vi "Single Tone Audio Measurements (N Ch).vi"(6 "units settings":T2, 8 "error in":errorcluster, 10 "measurement settings":T5={"Band start"=20.0, "Band stop"=20000.0, "Amplitude"=1.0, "Frequency"=1000.0, "Full scale range"=3.16}, 11 "waveforms":waveform(dbl)[](array[waveform])) -> (0 "error out":errorcluster, 1 "spectra":cluster{"x0":dbl, "dx":dbl, "magnitude":dbl[]}[](array[cluster]), 2 "waveforms":waveform(dbl)[](array[waveform]), 3 "results":T1[](array[typedef]))   [LabVIEW 2021]
uses:
  controls/single tone audio measurement settings.ctl
  controls/units settings.ctl
  controls/units - snr.ctl
  controls/units - ratio.ctl
  controls/single tone audio measurements.ctl
  <vilib>/addons/_NISVFA/_Shared subVIs/Common/SVL Set dB Reference (N Ch - 1 Ref).vi
  <vilib>/addons/Sound and Vibration/svt_Single Tone Measurements/SVT Spurious Free Dynamic Range (Frequency) (1 Ch).vi
  <vilib>/addons/_NISVFA/_Spectrum Processing/SVFA Unit Conversion (Complex) (1 Ch).vi
  <vilib>/addons/_NISVFA/_Shared subVIs/Common/SVL Set dB Reference (1 Ch).vi
  <vilib>/addons/_NISVFA/_Spectrum Processing/SVFA Get Spectrum Subset.vi
  <vilib>/addons/_NISVFA/_Spectrum Processing/SVFA Get Spectrum Subset (Complex) (1 Ch).vi
  <vilib>/addons/_NISVFA/_Shared subVIs/Common/svc_Window Parameters.vi
  <vilib>/addons/_NISVFA/_Shared subVIs/Common/svc_Extract Single Tone Information (complex).vi
  <vilib>/addons/_NISVFA/_Shared subVIs/Common/svc_Check Frequency Range in Spectrum.vi
  <vilib>/addons/_NISVFA/_Spectrum Processing/SVFA Spectrum Peak Search.vi
  <vilib>/addons/_NISVFA/_Spectrum Processing/SVFA Spectrum Peak Search (1 Ch).vi
  <vilib>/addons/_NISVFA/_Shared subVIs/Common/svc_Spectrum Units.vi
  <vilib>/addons/_NISVFA/_Shared subVIs/Common/svc_Log View for Spectrum (1Ch).vi
  <vilib>/addons/_NISVFA/_Spectrum Processing/SVFA Unit Conversion (1 Ch).vi
  <vilib>/addons/_NISVFA/_Shared subVIs/Common/svc_Complex Datatype Defaults.vi
  <vilib>/addons/_NISVFA/_Shared subVIs/Common/SVL Set dB Reference (variant).vi
  <vilib>/addons/_NISVFA/_Shared subVIs/Common/svc_Build Unit Label for Frequency Range.vi
  <vilib>/addons/_NISVFA/_Spectrum Processing/SVFA Get Tone Amplitude and Phase (1 Ch).vi
  <vilib>/addons/_NISVFA/_Spectrum Processing/subVIs/svfa_Compute Complex Spectrum for Export.vi
  <vilib>/addons/_NISVFA/_Shared subVIs/Common/svc_Check Frequency Range in Bandwidth.vi
  <vilib>/addons/_NISVFA/_Shared subVIs/Common/svc_Convert Start and Stop to Start Index and Length.vi
  <vilib>/addons/_NISVFA/_Spectrum Processing/subVIs/svfa_Spectrum Peak Search.vi
  <vilib>/addons/_NISVFA/_Shared subVIs/Common/svc_Format Value (DBL).vi
  <vilib>/addons/_NISVFA/_Shared subVIs/Common/svc_Get Weighting Enum and Labels.vi
  <vilib>/addons/_NISVFA/_Shared subVIs/Common/svc_Engineering Units to Unit Label.vi
  <vilib>/addons/_NISVFA/_Shared subVIs/Common/svc_Surround NonAlpha String with Parentheses.vi
  <vilib>/dlg_ctls.llb/Space Constant.vi
  <vilib>/addons/_NISVFA/_Shared subVIs/Common/svc_Unwrap Phase.vi
  <vilib>/addons/_NISVFA/_Shared subVIs/Common/svc_Convert Spectrum Array to dB.vi
  <vilib>/addons/_NISVFA/_Spectrum Processing/subVIs/svfa_Conversion Utility (spectrum info).vi
  <vilib>/addons/_NISVFA/_Spectrum Processing/subVIs/svfa_Window Frequency Response.vi
  <vilib>/addons/_NISVFA/_Spectrum Processing/subVIs/svfa_Window Frequency Response (double array).vi
  <vilib>/Analysis/baseanly.llb/Dot Product.vi
  <vilib>/Analysis/baseanly.llb/Complex Dot Product.vi
  <vilib>/addons/_NISVFA/_Spectrum Processing/subVIs/svfa_Peak Rough Search Indices.vi
  <vilib>/addons/_NISVFA/_Shared subVIs/Common/svc_Unit Label Lexical Class.vi
  <vilib>/addons/_NISVFA/_Spectrum Processing/subVIs/svfa_Peak to RMS to Peak2Peak.vi
  <vilib>/addons/_NISVFA/_Spectrum Processing/subVIs/svfa_Mag to Mag2.vi
  <vilib>/addons/_NISVFA/_Spectrum Processing/subVIs/svfa_Linear to dB.vi
  <vilib>/addons/_NISVFA/_Spectrum Processing/subVIs/svfa_dBrefA to dBrefB.vi
  <vilib>/addons/_NISVFA/_Spectrum Processing/subVIs/svfa_Spectrum to Spectral Density.vi
  <vilib>/addons/_NISVFA/_Spectrum Processing/subVIs/svfa_Rect Window Frequency Response.vi
  <vilib>/addons/_NISVFA/_Spectrum Processing/subVIs/svfa_Cosine Window Coefficients.vi
  <vilib>/addons/_NISVFA/_Shared subVIs/Common/svc_Caller VI Returned in Error Source.vi
  <vilib>/addons/Sound and Vibration/svt_Single Tone Measurements/SVT Gain (Time) (1 Ch).vi
  <vilib>/addons/Sound and Vibration/svt_Distortion/SVT SNR without Harmonics (Frequency) (1 Ch).vi
  <vilib>/addons/_NISVFA/_Spectrum Processing/SVFA Extract Single Tone Information (Complex) (1 Ch).vi
  <vilib>/addons/Sound and Vibration/svt_Single Tone Measurements/SVT Dynamic Range (Frequency) (1 Ch).vi
  <vilib>/addons/Sound and Vibration/svt_Distortion/subVIs/sv_Check Data Valid (Audio) (1 Ch).vi
  <vilib>/addons/_NISVFA/_Shared subVIs/Common/svc_Convert Frequency to Frequency String.vi
  <vilib>/Analysis/4window.llb/window parameters.vi
  <vilib>/Analysis/4window.llb/Window Properties.vi
  <vilib>/Analysis/4window.llb/Window Properties by Name.vi
  <vilib>/addons/_NISVFA/_Spectrum Processing/subVIs/svfa_Spectrum Peak Tone Search and Estimation (complex).vi
  <vilib>/measure/masignal.llb/Tones and Noise Waveform.vi
  <vilib>/addons/_NISVFA/_Shared subVIs/Common/svc_FFT with Window.vi
  <vilib>/Analysis/1siggen.llb/Square Wave.vi
  <vilib>/addons/_NISVFA/_Spectrum Processing/subVIs/svfa_Three Finger Peak Search.vi
  <vilib>/addons/Sound and Vibration/svt_Distortion/subVIs/sv_Peak View Amplitude (1 Ch).vi
  <vilib>/addons/Sound and Vibration/svt_Single Tone Measurements/SoundVib_SingleTone.lvlib
  <vilib>/addons/Sound and Vibration/svt_Distortion/SoundVib_Distortion.lvlib
  controls/audio controls.lvlib
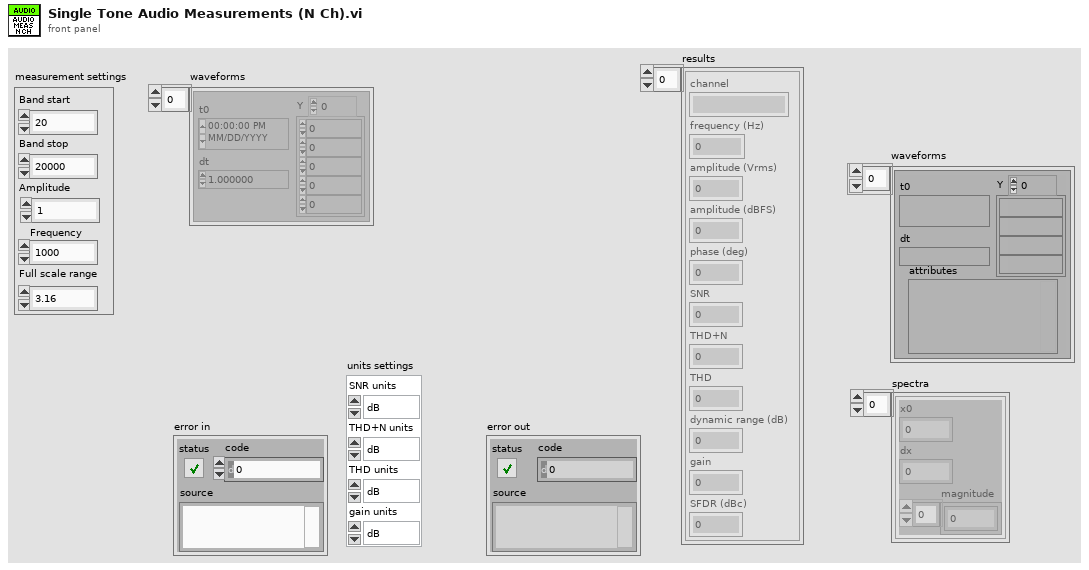
[diagram p1: front panel]
types:
  T1 = typedef "audio controls.lvlib/single tone audio measurements.ctl" = cluster{"channel":string, "frequency (Hz)":dbl, "amplitude (Vrms)":dbl, "amplitude (dBFS)":dbl, "phase (deg)":dbl, "SNR":dbl, "THD+N":dbl, "THD":dbl, "dynamic range (dB)":dbl, "gain":dbl, "SFDR (dBc)":dbl}
  T2 = typedef "audio controls.lvlib/units settings.ctl" = cluster{"SNR units":T3, "THD+N units":T4, "THD units":T4, "gain units":T4}
  T3 = typedef "audio controls.lvlib/units - snr.ctl" = enum32{"dB", "x/y"}
  T4 = typedef "audio controls.lvlib/units - ratio.ctl" = enum32{"dB", "%", "x/y"}
  T5 = typedef "single tone audio measurement settings.ctl" = cluster{"Band start":dbl, "Band stop":dbl, "Amplitude":dbl, "Frequency":dbl, "Full scale range":dbl}
  T6 = cluster{"start frequency":dbl, "stop frequency":dbl}
  T7 = cluster{"SNR units":enum16{"dB", "linear ratio", "%"}, "detected fundamental amplitude units":enum16{"EU rms", "EU peak", "EU peak-peak"}}
  T8 = cluster{"gain units":enum16{"dB", "linear ratio"}, "detected fundamental amplitude units":enum16{"EU rms", "EU peak", "EU peak-peak"}}
  T9 = enum16{"no change", "spectrum", "spectral density"}
  T10 = cluster{"linear/dB":enum16{"no change", "linear", "dB"}, "dB reference (0: no change)":dbl, "power/magnitude":enum16{"no change", "power", "magnitude"}, "view":enum16{"no change", "rms", "peak", "peak-peak"}}
  T11 = typedef "svc_Spectrum Info.ctl" = cluster{"channel name":string, "description":string, "x-axis units":T12, "spectral info":cluster{"spectrum type":T13, "linear/dB":enum16{"linear", "dB"}, "window":u16, "window size":i32, "FFT size":i32}, "engineering units":T14, "custom label":string, "dB reference [EU]":dbl, "peak units":enum16{"rms", "peak", "peak-peak"}, "weighting filter":T15, "spectral density?":bool, "unit label":string, "spectrum skewed?":bool, "complimentary spectrum units":T16}
  T12 = typedef "svc_X-Axis Units.ctl" = u16
  T13 = typedef "svc_Spectrum Type.ctl" = enum16{"FFT Spectrum [complex]", "Amplitude [Magnitude]", "Power [Magnitude^2]", "Cross Spectrum [complex]", "Frequency Response [Complex]"}
  T14 = typedef "svc_Engineering Units Text Ring.ctl" = u16
  T15 = typedef "svc_Weighting Filter Text Ring.ctl" = u16
  T16 = typedef "svc_Complimentary Spectrum Units.ctl" = enum16{"none", "radians", "degrees", "cycles", "imaginary"}
  T17 = cluster{"complex spectrum response":cluster{"f0":dbl, "df":dbl, "complex spectrum":cdb[]}, "spectrum info":T11}
  T18 = cluster{"frequency [Hz]":dbl, "amplitude [EU pk]":dbl, "phase (deg)":dbl}
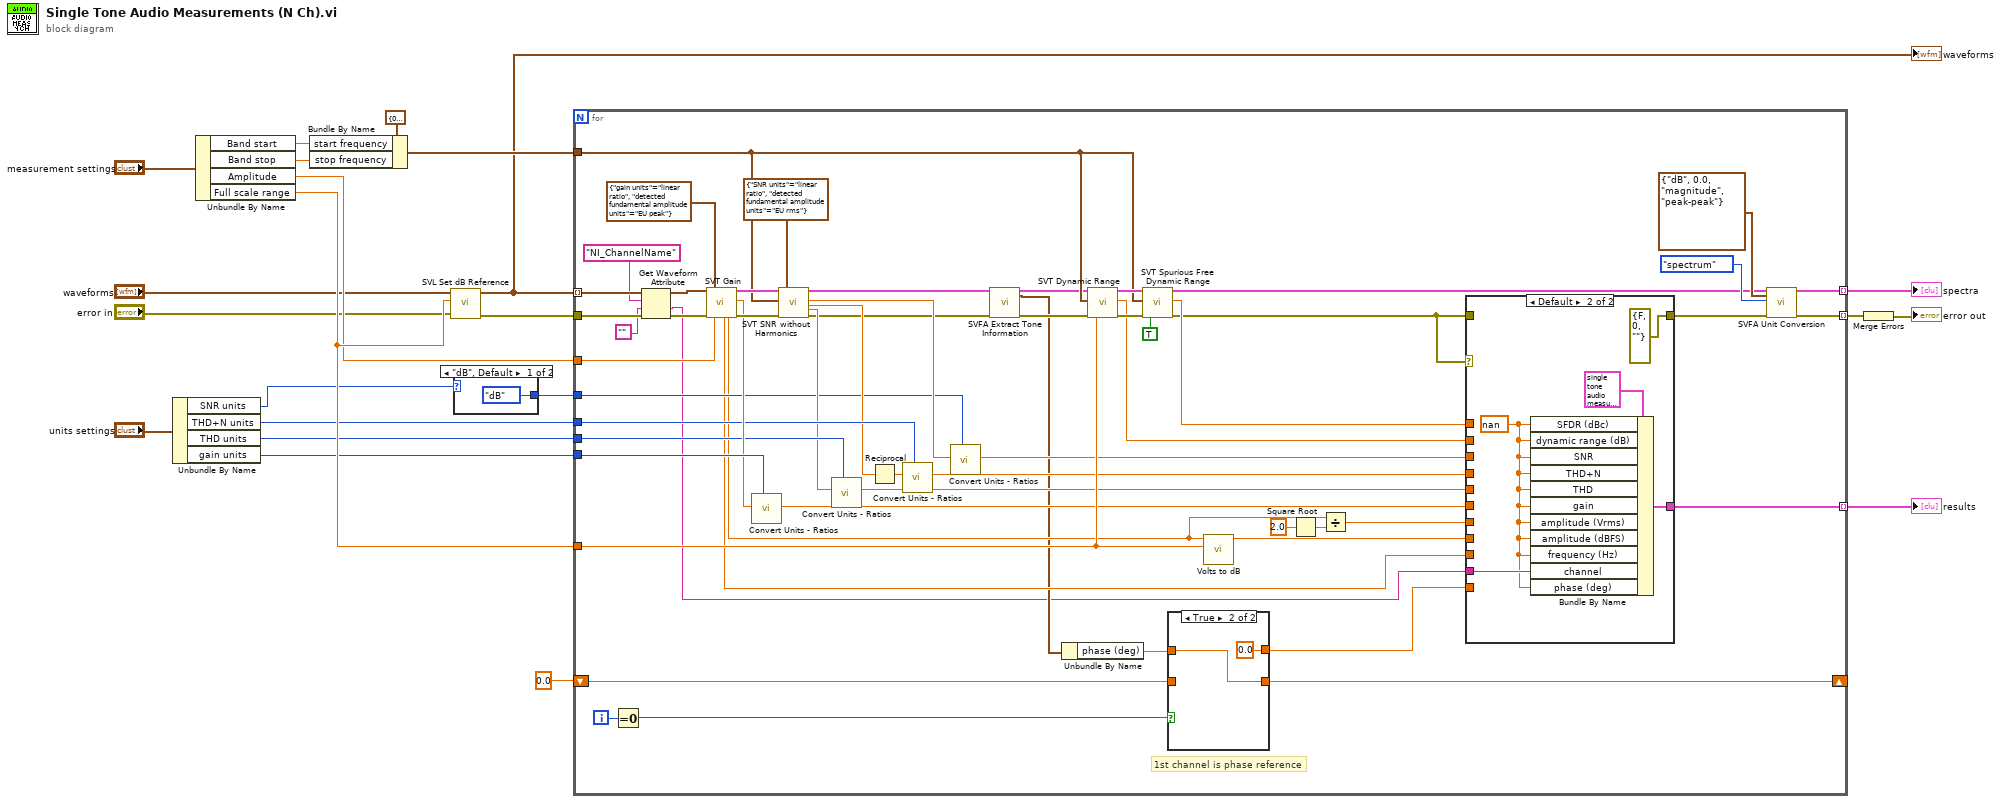
[diagram p0: block diagram]
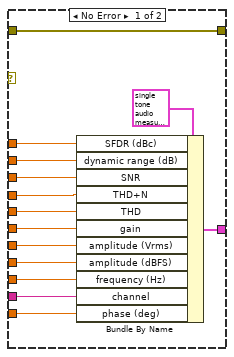
[diagram p2: hidden frame]
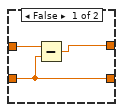
[diagram p3: hidden frame]
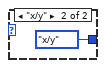
[diagram p4: hidden frame]
diagram:
  n1 = Unbundle By Name("units settings") -> ("SNR units"=w9:T3, "THD+N units"=w11:T4, "THD units"=w10:T4, "gain units"=w12:T4)
  n2 = Unbundle By Name("measurement settings") -> ("Band start"=w21:dbl, "Band stop"=w22:dbl, "Amplitude"=w15:dbl, "Full scale range"=w17:dbl)
  n3 = Bundle By Name(cluster=T6 {"start frequency"=0.0, "stop frequency"=0.0} ("frequency range"), "start frequency"=w21, "stop frequency"=w22) -> (w19:T6)
  n4 = call-poly <vilib>:"SVL Set dB Reference.vi"("error in (no error)"="error in", "dB reference [EU]"=w17, "scaled signals in [EU]"="waveforms") -> ("error out"=w16:errorcluster, "scaled signals out [EU]"=w6:waveform(dbl)[])  [unwired: 7 in]
  "waveforms" <- w6
  n5 = case shown="\"dB\", Default" w9 {
    tunnel: [units_-_ratio."dB" ("gain units") units_-_ratio."x/y" ("gain units")] -> w8
    frame "dB", Default {
    }
    frame "x/y" {
    }
  }
  n6 = for {
    tunnel: w19 -> [w72]
    tunnel: w17 -> [w71]
    tunnel: [w68] -> w4 mode=indexing
    tunnel: w15 -> [w67]
    tunnel: w12 -> [w66]
    tunnel: w11 -> [w63]
    tunnel: w10 -> [w57]
    tunnel: w8 -> [w54]
    tunnel: [w25] -> w3 mode=indexing
    tunnel: w6 -> [w36] mode=indexing
    shift-right: [w38] -> _
    shift-left: 0.0 -> [w40]
    tunnel: w16 -> [w34]
    tunnel: [w27] -> w1 mode=indexing
    i -> [w42]
    # "1st channel is phase reference"
    n7 = Equal To 0?(x=w42) -> (x = 0?=w41:bool)
    n8 = Get Waveform Attribute(4:w34, 5:"", 6:"NI_ChannelName" ("name"), 7:w36) -> (0:w33:errorcluster, 1:w30:string, 3:w35:waveform(dbl))  [unwired: 1 out]
    n9 = call-poly <vilib>:"SVT Gain.vi"("scaled signal [EU]"=w35, "error in (no error)"=w33, "desired units"=T8 {"gain units"=enum."linear ratio", "detected fundamental amplitude units"=enum."EU peak"}, "amplitude [EU peak]"=w67) -> ("detected fundamental\nfrequency [Hz]"=w53:dbl, "detected fundamental\namplitude"=w48:dbl, "complex spectrum"=w75:T17, "gain"=w65:dbl, "error out"=w76:errorcluster)  [unwired: 10 in, 1 out]
    n10 = call "Convert Units - Ratios.vi"("gain units"=w66, "linear ratio"=w65) -> ("converted ratio"=w64:dbl)  [unwired: 9 in]
    n11 = call-poly <vilib>:"SVT SNR without Harmonics.vi"("complex spectrum"=w75, "frequency range"=w72, "error in (no error)"=w76, "desired units"=T7 {"SNR units"=enum."linear ratio", "detected fundamental amplitude units"=enum."EU rms"}) -> ("complex spectrum"=w47:T17, "SNR (without harmonics)"=w62:dbl, "SINAD"=w59:dbl, "THD"=w56:dbl, "error out"=w46:errorcluster)  [unwired: 8 in, 3 out]
    n12 = call "Convert Units - Ratios.vi"("gain units"=w57, "linear ratio"=w56) -> ("converted ratio"=w55:dbl)  [unwired: 9 in]
    n13 = Reciprocal(x=w59) -> (1/x=w60:dbl)
    n14 = call "Convert Units - Ratios.vi"("gain units"=w63, "linear ratio"=w60) -> ("converted ratio"=w58:dbl)  [unwired: 9 in]
    n15 = call "Convert Units - Ratios.vi"("gain units"=w54, "linear ratio"=w62) -> ("converted ratio"=w61:dbl)  [unwired: 9 in]
    n16 = call-poly <vilib>:"SVFA Extract Tone Information.vi"("complex spectrum"=w47, "error in"=w46) -> ("complex spectrum"=w45:T17, "detected tone"=w43:T18, "error out"=w44:errorcluster)  [unwired: 14 in, 1 out]
    n17 = Unbundle By Name(w43) -> ("phase (deg)"=w39:dbl)
    n18 = call-poly <vilib>:"SVT Dynamic Range.vi"("complex spectrum"=w45, "frequency range"=w72, "error in (no error)"=w44, "full scale amplitude [EU peak]"=w71) -> ("dup complex spectrum"=w79:T17, "dynamic range"=w69:dbl, "error out"=w80:errorcluster)  [unwired: 10 in, 3 out]
    n19 = call-poly <vilib>:"SVT Spurious Free Dynamic Range.vi"("complex spectrum"=w79, "frequency range"=w72, "error in (no error)"=w80, "exclude harmonics"=TRUE) -> ("complex spectrum"=w26:T17, "spurious free dynamic range"=w70:dbl, "error out"=w29:errorcluster)  [unwired: 8 in, 5 out]
    n20 = case shown="True" w41 {
      tunnel: w40 -> [w102 _]
      tunnel: w39 -> [w103 w105]
      tunnel: [w101 0.0] -> w37
      tunnel: [w102 w105] -> w38
      frame False {
        n21 = Subtract(x=w103, y=w102) -> (x-y=w101:dbl)
      }
      frame True {
      }
    }
    n22 = call "Volts to dB.vi"("Full scale range"=w71, "Voltage(V)"=w48) -> ("Voltage(dB)"=w52:dbl)  [unwired: 9 in]
    n23 = Square Root(x=2.0 ("y")) -> (sqrt(x)=w51:dbl)
    n24 = Divide(x=w48, y=w51) -> (x/y=w49:dbl)
    n25 = case shown="Default" w29 {
      tunnel: w70 -> [w95 _]
      tunnel: w69 -> [w94 _]
      tunnel: [w92 w99] -> w68
      tunnel: w64 -> [w91 _]
      tunnel: w61 -> [w90 _]
      tunnel: w58 -> [w89 _]
      tunnel: w55 -> [w88 _]
      tunnel: w53 -> [w87 _]
      tunnel: w52 -> [w86 _]
      tunnel: w49 -> [w85 _]
      tunnel: w37 -> [w84 _]
      tunnel: w30 -> [w83 w98]
      tunnel: w29 -> [w82 _]
      tunnel: [w82 errorcluster {"status"=FALSE, "code"=0, "source"=""} ("error out")] -> w28
      frame No Error {
        n26 = Bundle By Name(cluster=T1 {"channel"="", "frequency (Hz)"=0.0, "amplitude (Vrms)"=0.0, "amplitude (dBFS)"=0.0, "phase (deg)"=0.0, "SNR"=0.0, "THD+N"=0.0, "THD"=0.0, "dynamic range (dB)"=0.0, "gain"=0.0, "SFDR (dBc)"=0.0} ("results"), "SFDR (dBc)"=w95, "dynamic range (dB)"=w94, "SNR"=w90, "THD+N"=w89, "THD"=w88, "gain"=w91, "amplitude (Vrms)"=w85, "amplitude (dBFS)"=w86, "frequency (Hz)"=w87, "channel"=w83, "phase (deg)"=w84) -> (w92:T1)
      }
      frame Default {
        w96 = nan ("SFDR (dBc)")
        n27 = Bundle By Name(cluster=T1 {"channel"="", "frequency (Hz)"=0.0, "amplitude (Vrms)"=0.0, "amplitude (dBFS)"=0.0, "phase (deg)"=0.0, "SNR"=0.0, "THD+N"=0.0, "THD"=0.0, "dynamic range (dB)"=0.0, "gain"=0.0, "SFDR (dBc)"=0.0} ("results"), "SFDR (dBc)"=w96, "dynamic range (dB)"=w96, "SNR"=w96, "THD+N"=w96, "THD"=w96, "gain"=w96, "amplitude (Vrms)"=w96, "amplitude (dBFS)"=w96, "frequency (Hz)"=w96, "channel"=w98, "phase (deg)"=w96) -> (w99:T1)
      }
    }
    n28 = call-poly <vilib>:"SVFA Unit Conversion.vi"("complex spectrum"=w26, "desired scaling"=T10 {"linear/dB"=enum."dB", "dB reference (0: no change)"=0.0, "power/magnitude"=enum."magnitude", "view"=enum."peak-peak"}, "spectral density desired"=T9."spectrum", "error in (no error)"=w28) -> ("converted spectrum"=w25:cluster{"x0":dbl, "dx":dbl, "magnitude":dbl[]}, "error out"=w27:errorcluster)  [unwired: 10 in, 4 out]
  }
  "results" <- w4
  "spectra" <- w3
  n29 = Merge Errors(w1) -> (→"error out":errorcluster)
